vi "DSS-test-readers.vi"(8 "error in":errorcluster) -> (0 "error out":errorcluster)   [LabVIEW 2020, in "DSS-Tests.lvlib"]
doc: "Caraya test of RFH-read-common_format and RFH-read-libreVNA: length, first and last element of every Common Format array against their golden files."
uses:
  DSS-Tests.lvlib
  <vilib>/addons/_JKI Toolkits/Caraya/classes/Test/Test.lvclass
  Reflector/RFH-Reflection_File_Handler.lvlib
  <vilib>/addons/_JKI Toolkits/Caraya/classes/Assert/Assert.lvclass
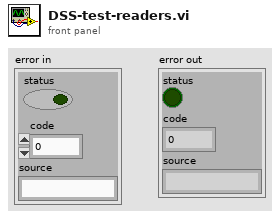
[diagram p1: front panel]
types:
  T1 = typedef "RFH-Reflection_File_Handler.lvlib/RFH-common_data_format.ctl" = cluster{"Frequency":dbl[], "Reflection'":dbl[], "Reflection''":dbl[], "Permativity'":dbl[], "Permativity''":dbl[], "Conductivity":dbl[], "Loss Tangent":dbl[], "Resistance":dbl[], "Reactance":dbl[]}
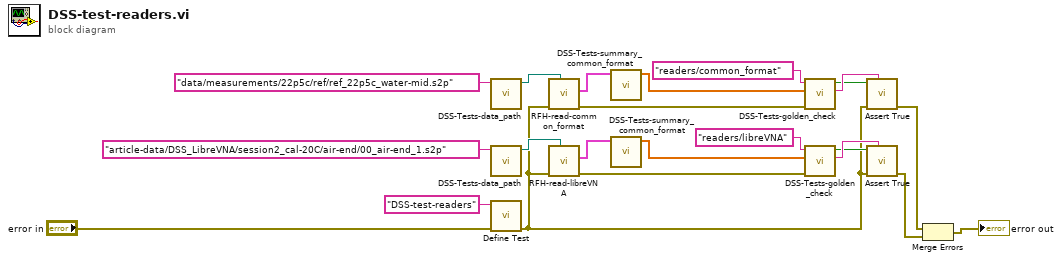
[diagram p0: block diagram]
diagram:
  n1 = call "DSS-Tests-data_path.vi"("relative path"="data/measurements/22p5c/ref/ref_22p5c_water-mid.s2p") -> ("path"=w5:path)  [unwired: 10 in]
  n2 = call "DSS-Tests-data_path.vi"("relative path"="article-data/DSS_LibreVNA/session2_cal-20C/air-end/00_air-end_1.s2p") -> ("path"=w14:path)  [unwired: 10 in]
  n3 = call <vilib>:"Define Test.vi"("error in (no error)"="error in", "Label (VI Title)"="DSS-test-readers") -> ("error out"=w3:errorcluster)  [unwired: 8 in, 1 out]
  n4 = call "RFH-read-common_format.vi"("file path (dialog if empty)"=w5, "error in"=w3) -> ("error out"=w6:errorcluster, "Common Format"=w7:T1)  [unwired: 8 in]
  n5 = call "RFH-read-libreVNA.vi"("file path (dialog if empty)"=w14, "error in"=w3) -> ("error out"=w15:errorcluster, "Common Format"=w16:T1)  [unwired: 8 in]
  n6 = call "DSS-Tests-summary_common_format.vi"("Common Format"=w7) -> ("summary"=w8:dbl[])  [unwired: 10 in]
  n7 = call "DSS-Tests-summary_common_format.vi"("Common Format"=w16) -> ("summary"=w17:dbl[])  [unwired: 10 in]
  n8 = call "DSS-Tests-golden_check.vi"("error in"=w6, "actual"=w8, "golden name"="readers/common_format") -> ("message"=w11:string, "pass"=w10:bool)  [unwired: 6 in, 1 out]
  n9 = call "DSS-Tests-golden_check.vi"("error in"=w15, "actual"=w17, "golden name"="readers/libreVNA") -> ("message"=w20:string, "pass"=w19:bool)  [unwired: 6 in, 1 out]
  n10 = call <vilib>:"Assert True.vi"("Label"=w11, "error in (no error)"=w3, "True?"=w10) -> ("error out"=w12:errorcluster)  [unwired: 7 in, 1 out]
  n11 = call <vilib>:"Assert True.vi"("Label"=w20, "error in (no error)"=w3, "True?"=w19) -> ("error out"=w21:errorcluster)  [unwired: 7 in, 1 out]
  n12 = Merge Errors(w12, w21) -> (→"error out":errorcluster)
